vi "Show.vi"(8 "error in (no error)":errorcluster, 11 "ToastFromXML in":refnum<class "ToastFromXML.lvclass">) -> (0 "error out":errorcluster, 3 "ToastFromXML out":refnum<class "ToastFromXML.lvclass">)   [LabVIEW 2026, in "ToastNotification.lvlib" / "ToastFromXML.lvclass"]
doc: "Display the retained XML Document as a Windows toast. Skipped on incoming error. ToastService.Show invokes this ToastSource override. Creates and releases temporary notification and notifier references; keeps the document alive for reuse. Callback registration is separate and the caller still owns Close."
uses:
  ToastFromXML.lvclass
  ToastFromXML.lvclass/ToastFromXML.ctl
  Read XML Document.vi
  Toast Native/Toast Native.lvlib
  Reflection DotNet/Reflection DotNet.lvlib
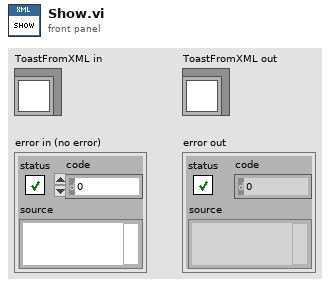
[diagram p1: front panel]
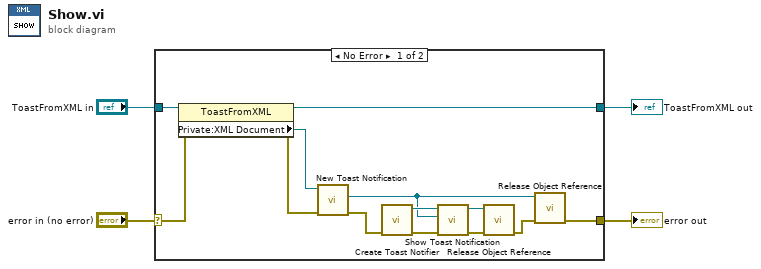
[diagram p0: block diagram]
diagram:
  n1 = case shown="No Error" "error in (no error)" {
    selector: "error in (no error)" -> [w15 w18]
    tunnel: "ToastFromXML in" -> [w17 w19]
    tunnel: [w16 w19] -> w2
    tunnel: [w6 w18] -> w1
    frame No Error {
      n2 = property class="ToastFromXML"(reference=w17, error in=w15) -> (reference out=w16:refnum<class "ToastFromXML.lvclass">, error out=w5:errorcluster, "Private:XML Document"=w14:refnum<k24>)
      n3 = call "New Toast Notification.vi"("error in"=w5, "XML Document in"=w14) -> ("error out"=w12:errorcluster, "Toast Notification"=w8:refnum<k24>)  [unwired: 7 in, 1 out]
      n4 = call "Create Toast Notifier.vi"("error in"=w12) -> ("error out"=w13:errorcluster, "Toast Notifier"=w11:refnum<k24>)  [unwired: 9 in]
      n5 = call "Show Toast Notification.vi"("error in"=w13, "Toast Notification"=w8, "Toast Notifier in"=w11) -> ("error out"=w10:errorcluster, "Toast Notifier out"=w9:refnum<k24>)  [unwired: 7 in]
      n6 = call "Release Object Reference.vi"("error in"=w10, "object"=w9) -> ("error out"=w7:errorcluster)  [unwired: 9 in]
      n7 = call "Release Object Reference.vi"("error in"=w7, "object"=w8) -> ("error out"=w6:errorcluster)  [unwired: 9 in]
    }
    frame Error {
    }
  }
  "error out" <- w1
  "ToastFromXML out" <- w2
